vi "Build Resistor Ciphers.vi"(8 "error in (no error)":errorcluster, 10 "Number of Bands":T6=4 min=3 max=6 step=1, 11 "Selectors":T1={"1Dig"=enum."Black - 0", "2Dig"=enum."Black - 0", "3Dig"=enum."Black - 0", "Mul"=enum."Silver - x 0.01", "Tol"=enum."Gold - 5%", "TC"=enum."Grey - 1 ppm/K"}) -> (0 "error out":errorcluster, 2 "Negative":bool, 3 "Nominal Value":i32)   [LabVIEW 2018, in "Resistance Value.lvlib"]
doc: "Builds the Ciphers array used to calculate the resistor significant value according to the selected number of bands.\n\nThe VI receives the <b>Selectors</b> cluster, containing the selected values for the first, second, and third significant digits, and the <b>Number of Bands</b>.\n\nFor 3- and 4-band resistors, the resistor has two significant digits. The resulting Ciphers array is built as:\n\n[0, 1st Digit, 2nd Digit]\n\nFor 5- and 6-band resistors, the resistor has three significant digits. The resulting Ciphers array is built as:\n\n[1st Digit, 2nd Digit, 3rd Digit]\n\nThe resulting Ciphers array is passed to <b>Cipher to Number.vi</b>, which calculates the corresponding integer value.\n\nThe VI returns the resulting value through <b>Nominal Value</b>, indicates whether the value is negative through <b>Negative</b>, and propagates errors through <b>error in</b> and <b>error out</b>."
uses:
  Resistance Value.lvlib
  Number of Bands--numeric.ctl
  Resistor Controls/Selectors--cluster.ctl
  Resistor Controls/Digit--enum.ctl
  Resistor Controls/Multiplier--enum.ctl
  Resistor Controls/Tolerance--enum.ctl
  Resistor Controls/Temp Coefficient--enum.ctl
  Resistor Controls/Resistance Controls.lvlib
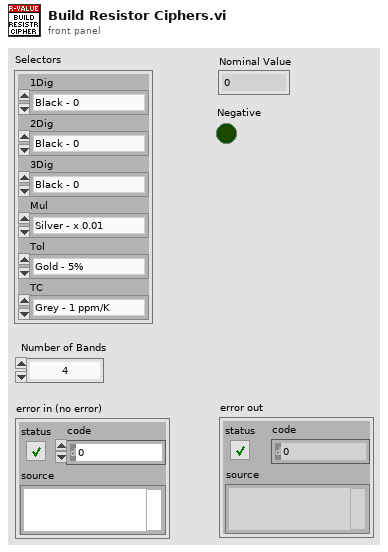
[diagram p1: front panel]
types:
  T1 = typedef "Resistance Controls.lvlib/Selectors--cluster.ctl" = cluster{"1Dig":T2, "2Dig":T2, "3Dig":T2, "Mul":T3, "Tol":T4, "TC":T5}
  T2 = typedef "Resistance Controls.lvlib/Digit--enum.ctl" = enum16{"Black - 0", "Brown - 1", "Red - 2", "Orange - 3", "Yellow - 4", "Green - 5", "Blue - 6", "Violet - 7", "Grey - 8", "White - 9"}
  T3 = typedef "Resistance Controls.lvlib/Multiplier--enum.ctl" = enum16{"Silver - x 0.01", "Gold - x 0.1 ", "Black - x 1", "Brown - x 10", "Red - x 100", "Orange - x 1k", "Yellow - x 10k", "Green - 100k", "Blue - x 1M", "Violet - x10 M", "Grey - x 100M", "White - x 1G"}
  T4 = typedef "Resistance Controls.lvlib/Tolerance--enum.ctl" = enum16{"Gray - 0.05%", "Violet - 0.1%", "Blue - 0.25%", "Green - 0.5%", "Brown - 1%", "Red - 2%", "Gold - 5%", "Silver - 10%", "None - 20%"}
  T5 = typedef "Resistance Controls.lvlib/Temp Coefficient--enum.ctl" = enum16{"Grey - 1 ppm/K", "Violet - 5 ppm/K", "Blue - 10 ppm/K", "Green - 20 ppm/K", "Yellow - 25 ppm/K", "Orange - 15 ppm/K", "Red - 50 ppm/K", "Brown - 100 ppm/K", "Black - 250 ppm/K"}
  T6 = typedef "Number of Bands--numeric.ctl" = u8
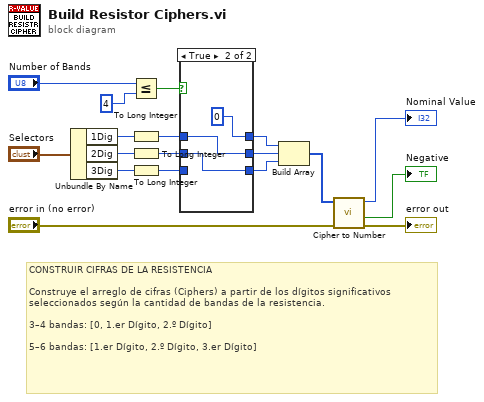
[diagram p0: block diagram]
diagram:
  # "CONSTRUIR CIFRAS DE LA RESISTENCIA\n\nConstruye el arreglo de cifras (Ciphers) a partir de los dígitos significativos seleccionados según la cantidad de bandas de la resistencia.\n\n3–4 bandas: [0, 1.er Dígito, 2.º Dígito]\n\n5–6 bandas: [1.er Dígito, 2.º Dígito, 3.er Dígito]"
  n1 = Unbundle By Name("Selectors") -> ("1Dig"=w2:T2, "2Dig"=w3:T2, "3Dig"=w1:T2)
  n2 = Less Or Equal?(x="Number of Bands", y=T6 4) -> (x <= y?=w11:bool)
  n3 = To Long Integer(number=w2) -> (32bit integer=w10:i32)
  n4 = To Long Integer(number=w3) -> (32bit integer=w9:i32)
  n5 = To Long Integer(number=w1) -> (32bit integer=w8:i32)
  n6 = case shown="True" w11 {
    tunnel: w10 -> [w21 w23]
    tunnel: w9 -> [w20 w24]
    tunnel: w8 -> [w19 _]
    tunnel: [w21 0] -> w7
    tunnel: [w20 w23] -> w6
    tunnel: [w19 w24] -> w5
    frame False {
    }
    frame True {
    }
  }
  n7 = Build Array(w7, w6, w5) -> (w12:i32[])
  n8 = call "Cipher to Number.vi"("error in (no error)"="error in (no error)", "Ciphers"=w12) -> ("error out"=→"error out":errorcluster, "Negative"=→"Negative":bool, "Number"=→"Nominal Value":i32)  [unwired: 7 in]
